vi "Game_Hover.vi"(0 "Context":T1={"Screen"=enum."Settings", "Settings"=[0, 0, 1, 1], "Board"={"Grid"=array15x15[225 elements], "Move History"=[], "Last Move"={"Row"=-1, "Col"=-1, "Stone"=enum."Empty"}}, "Status"=enum."Idle", "Game ID"=0, "Player Stone"=enum."Black", "Hover"={"Row"=-1, "Col"=-1, "Stone"=enum."Empty"}, "Hover Button"=-1, "Win Line"=[], "Score 1"=0, "Score 2"=0, "Draws"=0, "Status Text"="", "Status Color"=0}, 5 "X":i32, 7 "Y":i32, 11 "error in":errorcluster) -> (4 "Context out":T1={"Screen"=enum."Settings", "Settings"=[0, 0, 1, 1], "Board"={"Grid"=array15x15[225 elements], "Move History"=[], "Last Move"={"Row"=-1, "Col"=-1, "Stone"=enum."Empty"}}, "Status"=enum."Idle", "Game ID"=0, "Player Stone"=enum."Black", "Hover"={"Row"=-1, "Col"=-1, "Stone"=enum."Empty"}, "Hover Button"=-1, "Win Line"=[], "Score 1"=0, "Score 2"=0, "Draws"=0, "Status Text"="", "Status Color"=0}, 6 "Changed":bool, 15 "error out":errorcluster)   [LabVIEW 2026]
doc: "마우스 이동 (X,Y): 버튼 강조(Hover Button)와 바둑판 미리보기(Hover)를 갱신. Changed = 다시 그릴 필요."
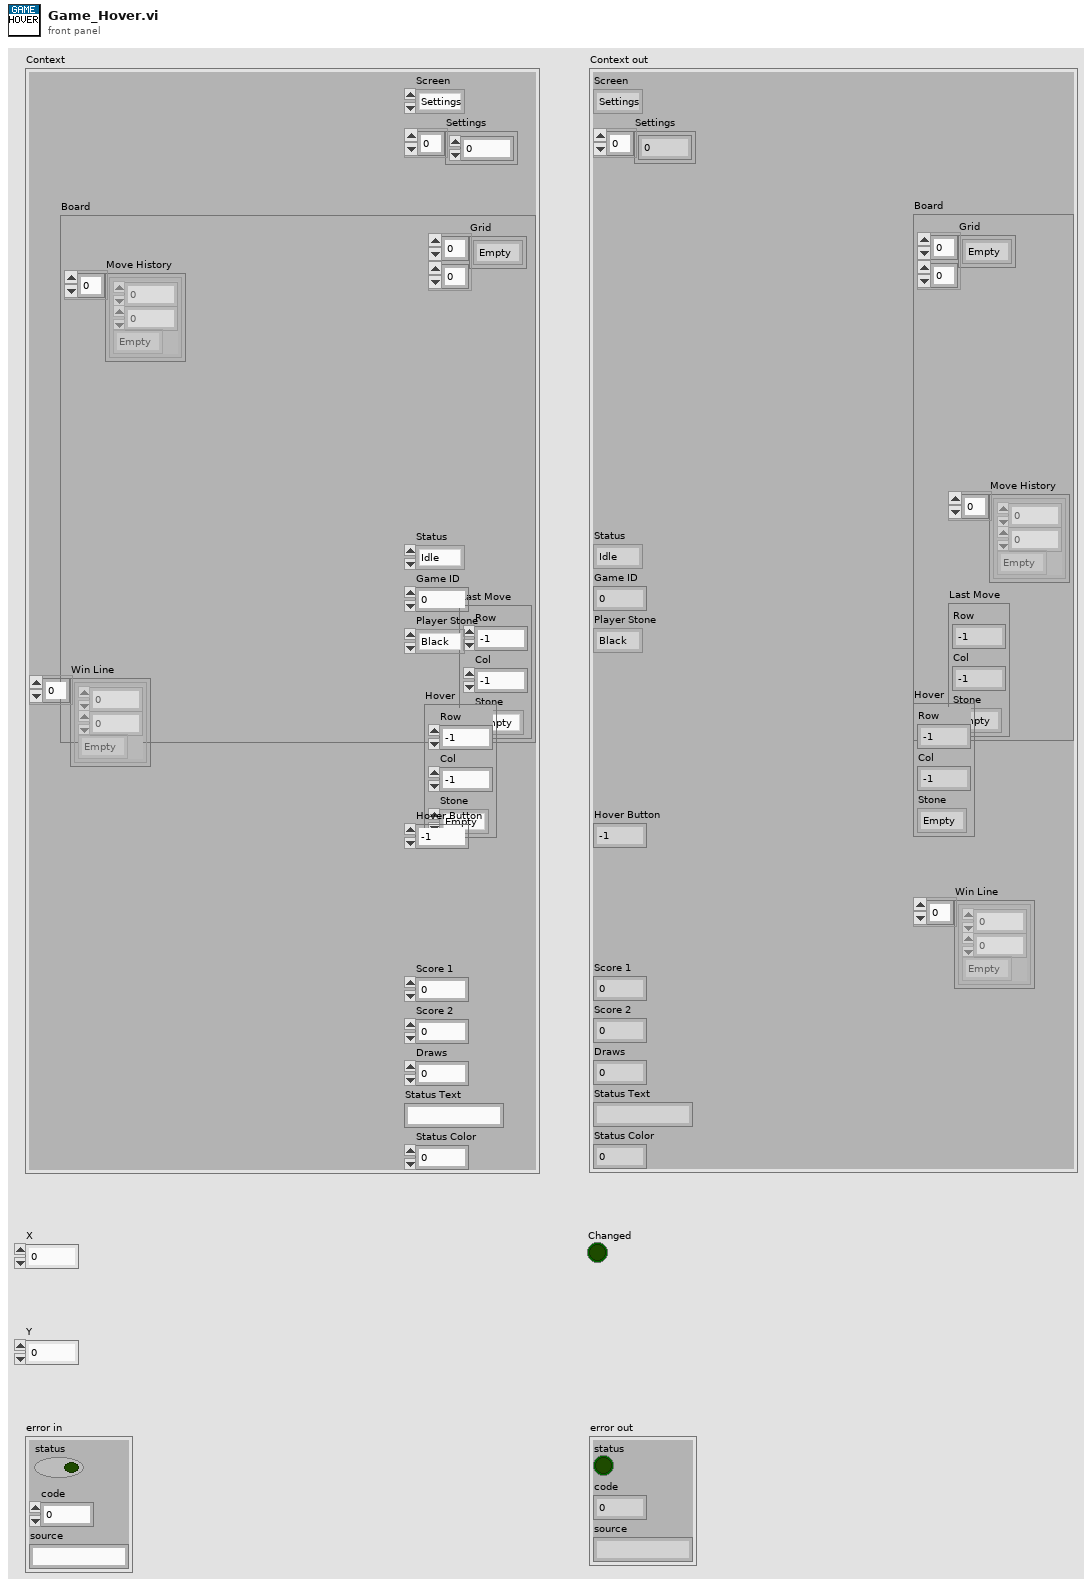
[diagram p1: front panel]
types:
  T1 = cluster{"Screen":enum16{"Settings", "Game"}, "Settings":i32[], "Board":cluster{"Grid":enum8{"Empty", "Black", "White"}[][], "Move History":cluster{"Row":i32, "Col":i32, "Stone":enum8{"Empty", "Black", "White"}}[], "Last Move":cluster{"Row":i32, "Col":i32, "Stone":enum8{"Empty", "Black", "White"}}}, "Status":enum16{"Idle", "Player Turn", "AI Thinking", "Game Over"}, "Game ID":u32, "Player Stone":enum8{"Empty", "Black", "White"}, "Hover":cluster{"Row":i32, "Col":i32, "Stone":enum8{"Empty", "Black", "White"}}, "Hover Button":i32, "Win Line":cluster{"Row":i32, "Col":i32, "Stone":enum8{"Empty", "Black", "White"}}[], "Score 1":i32, "Score 2":i32, "Draws":i32, "Status Text":string, "Status Color":u32}
  T2 = cluster{"Row":i32, "Col":i32, "Stone":enum8{"Empty", "Black", "White"}}
  T3 = enum16{"Idle", "Player Turn", "AI Thinking", "Game Over"}
  T4 = cluster{"Rect":cluster{"left":i16, "top":i16, "right":i16, "bottom":i16}, "Fill":u32, "Fill Sel":u32, "Border":u32, "Border Sel":u32, "Text":string, "Text Color":u32, "Text Sel":u32, "Size":i16, "Bold":bool, "Group":i32, "Value":i32, "Radius":i16}[]
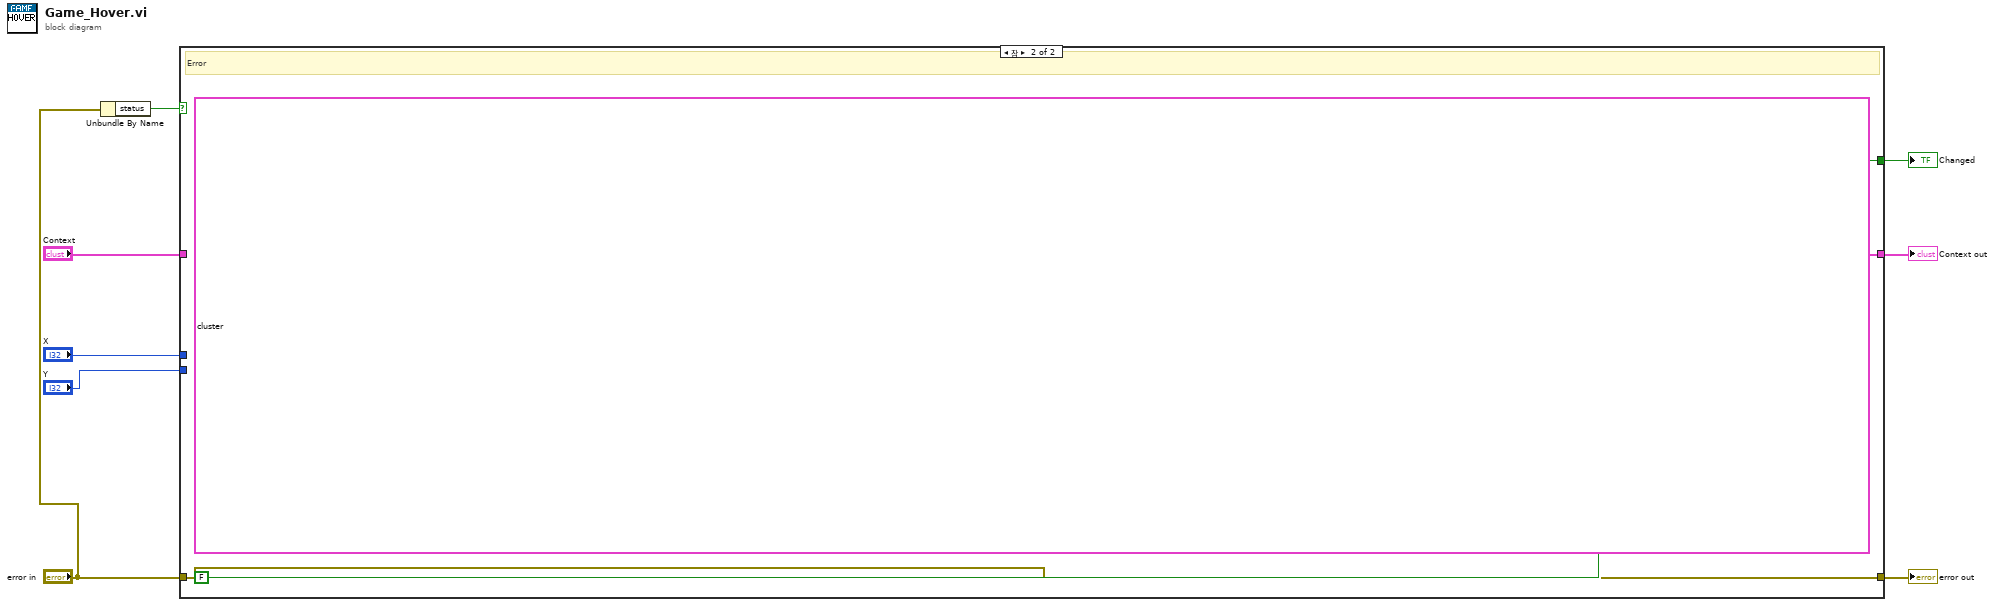
[diagram p0: block diagram]
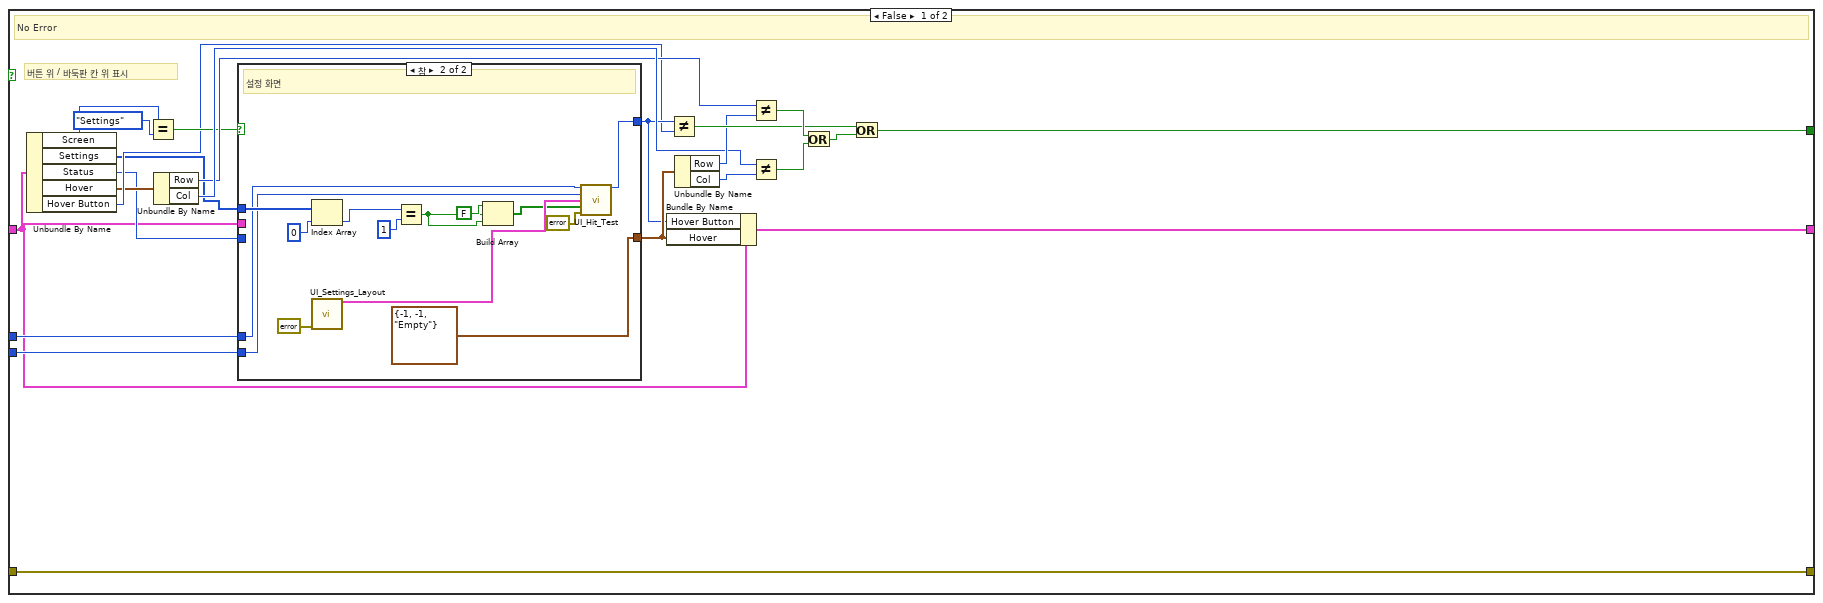
[diagram p2: hidden frame]
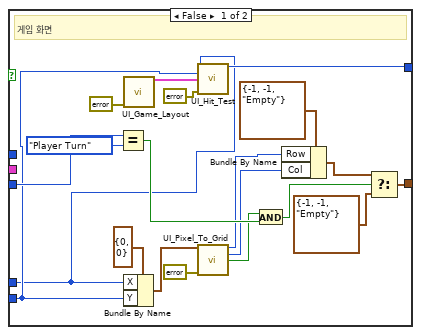
[diagram p3: hidden frame]
diagram:
  n1 = Unbundle By Name("error in") -> ("status"=w5:bool)
  n2 = case shown="참" w5 {
    tunnel: "Context" -> [w9 _]
    tunnel: "X" -> [w10 _]
    tunnel: "Y" -> [w11 _]
    tunnel: "error in" -> [w12 w66]
    tunnel: [w12 w66] -> w8
    tunnel: [w31 T1 {"Screen"=enum."Settings", "Settings"=[0, 0, 1, 1], "Board"={"Grid"=array15x15[225 elements], "Move History"=[], "Last Move"={"Row"=-1, "Col"=-1, "Stone"=enum."Empty"}}, "Status"=enum."Idle", "Game ID"=0, "Player Stone"=enum."Black", "Hover"={"Row"=-1, "Col"=-1, "Stone"=enum."Empty"}, "Hover Button"=-1, "Win Line"=[], "Score 1"=0, "Score 2"=0, "Draws"=0, "Status Text"="", "Status Color"=0}] -> w6
    tunnel: [w30 FALSE] -> w7
    frame False {
      # "버튼 위 / 바둑판 칸 위 표시"
      # "No Error"
      n3 = Unbundle By Name(w9) -> ("Screen"=w13:enum16{"Settings", "Game"}, "Settings"=w14:i32[], "Status"=w15:T3, "Hover"=w16:T2, "Hover Button"=w17:i32)
      n4 = Equal?(x=w13, y=enum16{"Settings", "Game"}."Settings") -> (x = y?=w19:bool)
      n5 = Unbundle By Name(w16) -> ("Row"=w22:i32, "Col"=w23:i32)
      n6 = case shown="참" w19 {
        tunnel: [w51 T2 {"Row"=-1, "Col"=-1, "Stone"=enum."Empty"}] -> w21
        tunnel: w9 -> [_ _]
        tunnel: w10 -> [w32 w52]
        tunnel: w11 -> [w33 w53]
        tunnel: w14 -> [_ w54]
        tunnel: w15 -> [w34 _]
        tunnel: [w38 w64] -> w20
        frame False {
          # "게임 화면"
          n7 = Equal?(x=w34, y=T3."Player Turn") -> (x = y?=w46:bool)
          n8 = call "UI_Game_Layout.vi"("error in"=errorcluster {"status"=FALSE, "code"=0, "source"=""}) -> ("Specs"=w36:T4)  [unwired: 13 in, 1 out]
          n9 = Bundle By Name(cluster=cluster{"X":i32, "Y":i32} {"X"=0, "Y"=0}, "X"=w32, "Y"=w33) -> (w40:cluster{"X":i32, "Y":i32})
          n10 = call "UI_Hit_Test.vi"("X"=w32, "Y"=w33, "Specs"=w36, "error in"=errorcluster {"status"=FALSE, "code"=0, "source"=""}) -> ("Index"=w38:i32)  [unwired: 8 in, 3 out]
          n11 = call "UI_Pixel_To_Grid.vi"("Coords"=w40, "error in"=errorcluster {"status"=FALSE, "code"=0, "source"=""}) -> ("Row"=w42:i32, "Col"=w43:i32, "Valid"=w44:bool)  [unwired: 10 in, 1 out]
          n12 = And(x=w44, y=w46) -> (x .and. y?=w47:bool)
          n13 = Bundle By Name(cluster=T2 {"Row"=-1, "Col"=-1, "Stone"=enum."Empty"}, "Row"=w42, "Col"=w43) -> (w49:T2)
          n14 = Select(t=w49, s=w47, f=T2 {"Row"=-1, "Col"=-1, "Stone"=enum."Empty"}) -> (s? t:f=w51:T2)
        }
        frame True {
          # "설정 화면"
          n15 = Index Array(array=w54, index=0) -> (element=w56:i32)
          n16 = call "UI_Settings_Layout.vi"("error in"=errorcluster {"status"=FALSE, "code"=0, "source"=""}) -> ("Specs"=w62:T4)  [unwired: 13 in, 1 out]
          n17 = Equal?(x=w56, y=1) -> (x = y?=w58:bool)
          n18 = Build Array(FALSE, w58, w58) -> (w60:bool[])
          n19 = call "UI_Hit_Test.vi"("X"=w52, "Y"=w53, "Specs"=w62, "Dim Groups"=w60, "error in"=errorcluster {"status"=FALSE, "code"=0, "source"=""}) -> ("Index"=w64:i32)  [unwired: 7 in, 3 out]
        }
      }
      n20 = Bundle By Name(cluster=w9, "Hover Button"=w20, "Hover"=w21) -> (w31:T1)
      n21 = Not Equal?(x=w20, y=w17) -> (x != y?=w26:bool)
      n22 = Unbundle By Name(w21) -> ("Row"=w24:i32, "Col"=w25:i32)
      n23 = Not Equal?(x=w22, y=w24) -> (x != y?=w27:bool)
      n24 = Not Equal?(x=w23, y=w25) -> (x != y?=w28:bool)
      n25 = Or(x=w27, y=w28) -> (x .or. y?=w29:bool)
      n26 = Or(x=w26, y=w29) -> (x .or. y?=w30:bool)
    }
    frame True {
      # "Error"
    }
  }
  "Context out" <- w6
  "Changed" <- w7
  "error out" <- w8
